vi "VI Name Generation.vi"(11 "Test Case In":refnum<class "Generate VI Names.lvclass">) -> (0 "error out":errorcluster, 3 "Test Case Out":refnum<class "Generate VI Names.lvclass">)   [LabVIEW 2026, in "Generate VI Names.lvclass"]
doc: "Test creation of labview styled VI names from python compatible function names."
uses:
  Generate VI Names.lvclass
  Generate VI Names.lvclass/Generate VI Names.ctl
  <vilib>/Astemes/LUnit/Test Case.lvclass/Test Case.ctl
  4993e8ee-a06a-463a-9684-69129f64d5ce.vi
  <vilib>/Astemes/LUnit/Core/LUnit Test Case/Private/Append Pass Result.vi
  <vilib>/Astemes/LUnit/Core/LUnit Test Case/Private/Append Fail Result.vi
  4993e8ee-a06a-463a-9684-69129f64d5ce.vi/9c5d11cd-9439-4240-a1ee-d9baace9c924.vi
  <vilib>/Astemes/LUnit/Core/LUnit Test Case/Private/Run In UI.vi
  <vilib>/Utility/error.llb/Clear Errors.vi
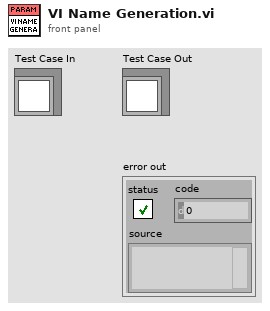
[diagram p1: front panel]
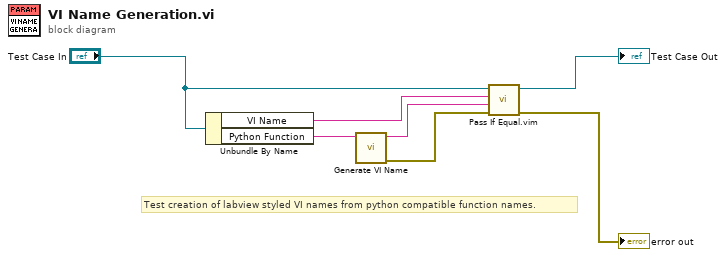
[diagram p0: block diagram]
diagram:
  # "Test creation of labview styled VI names from python compatible function names."
  n1 = Unbundle By Name("Test Case In") -> ("VI Name"=w3:string, "Python Function"=w2:string)
  n2 = call "Generate VI Name.vi"("Python Function Name"=w2) -> ("error out"=w6:errorcluster, "VI Name"=w1:string)  [unwired: 9 in]
  n3 = call "Pass If Equal.vim"("error in (no error)"=w6, "Actual"=w1, "Expected"=w3, "LUnit Test Case In"="Test Case In") -> ("error out"=→"error out":errorcluster, "LUnit Test Case Out"=→"Test Case Out":refnum<class "Generate VI Names.lvclass">)  [unwired: 6 in]
